vi "Build_Asylum_SetPISLoop.vi"(6 "outChannelString":string, 7 "whichLoop":i32, 8 "error in (no error)":errorcluster, 9 "PIS Controls":T1, 10 "inChannelString":string, 11 "eventString":string) -> (0 "error out":errorcluster, 3 "Command":string)   [LabVIEW 2019]
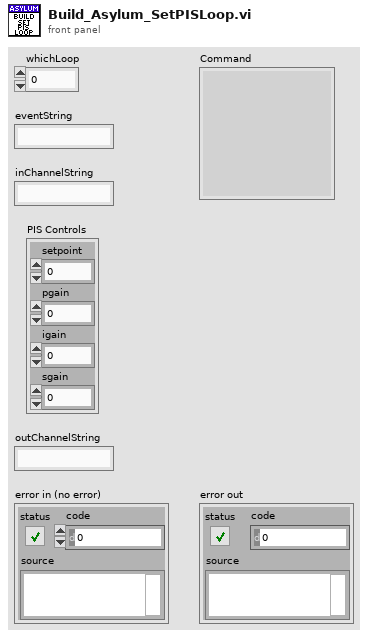
[diagram p1: front panel]
types:
  T1 = cluster{"setpoint":dbl, "pgain":dbl, "igain":dbl, "sgain":dbl}
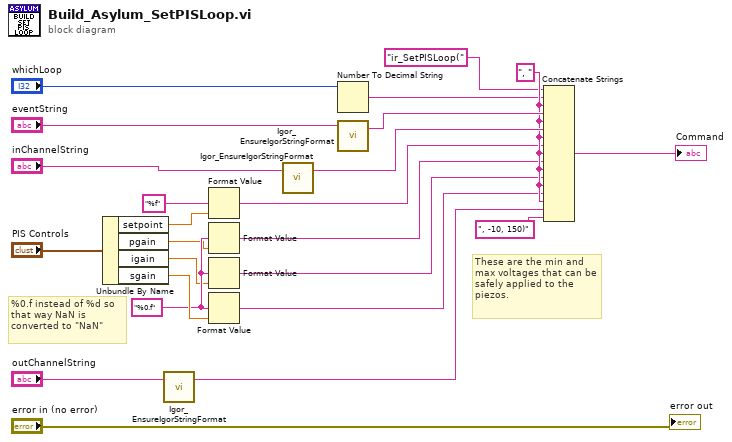
[diagram p0: block diagram]
diagram:
  w10 = "%0.f" ("format string")
  w19 = ", " ("string")
  # "%0.f instead of %d so that way NaN is converted to \"NaN\""
  # "These are the min and max voltages that can be safely applied to the piezos."
  n1 = Unbundle By Name("PIS Controls") -> ("setpoint"=w3:dbl, "pgain"=w8:dbl, "igain"=w9:dbl, "sgain"=w11:dbl)
  n2 = call <userlib>:"Igor_EnsureIgorStringFormat.vi"("Value"="outChannelString") -> ("Value"=w24:string)  [unwired: 2 in]
  n3 = Format Value(format string="%f" ("Expected output Format"), value (0)=w3) -> (output string=w7:string)  [unwired: 1 in]
  n4 = Format Value(format string=w10, value (0)=w8) -> (output string=w6:string)  [unwired: 1 in]
  n5 = Format Value(format string=w10, value (0)=w9) -> (output string=w5:string)  [unwired: 1 in]
  n6 = Format Value(format string=w10, value (0)=w11) -> (output string=w4:string)  [unwired: 1 in]
  n7 = call <userlib>:"Igor_EnsureIgorStringFormat.vi"("Value"="inChannelString") -> ("Value"=w23:string)  [unwired: 2 in]
  n8 = Number To Decimal String(number="whichLoop") -> (decimal integer string=w15:string)  [unwired: 1 in]
  n9 = call <userlib>:"Igor_EnsureIgorStringFormat.vi"("Value"="eventString") -> ("Value"=w22:string)  [unwired: 2 in]
  n10 = Concatenate Strings("ir_SetPISLoop(" ("string"), w15, w19, w22, w19, w23, w19, w7, w19, w6, w19, w5, w19, w4, w19, w24, ", -10, 150)" ("string")) -> (→"Command":string)
  "error out" <- "error in (no error)"
